vi "Serialize Properties.vi"(8 "error in (no error)":errorcluster, 10 "Properties":refnum<class "Property.lvclass">[](array[class]), 11 "Node in":refnum<k20>) -> (0 "error out":errorcluster, 3 "Node out":refnum<k20>)   [LabVIEW 2013, in "JUnit XML.lvlib" / "Test Suite.lvclass"]
uses:
  Test Suite.lvclass
  <vilib>/xml/NI_XML.lvlib
  JUnit XML.lvlib
  <vilib>/xml/Close Reference(Node).vi
  Property/Property.lvclass
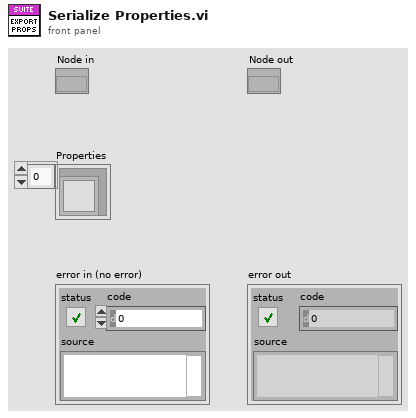
[diagram p1: front panel]
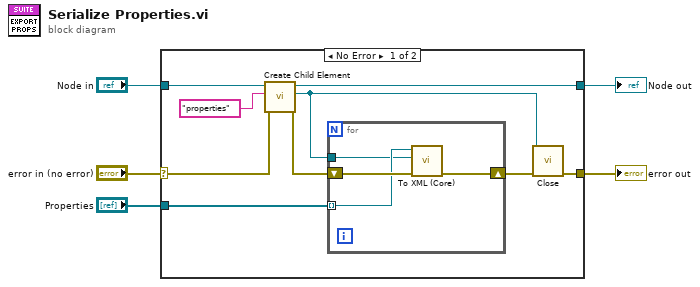
[diagram p0: block diagram]
diagram:
  n1 = case shown="No Error" "error in (no error)" {
    selector: "error in (no error)" -> [w7 w20]
    tunnel: "Node in" -> [w14 w19]
    tunnel: [w12 w20] -> w4
    tunnel: [w11 w19] -> w3
    tunnel: "Properties" -> [w9 _]
    frame No Error {
      n2 = call "Create Child Element.vi"("error in (no error)"=w7, "Name"="properties" ("Tag Name"), "Node in"=w14) -> ("error out"=w10:errorcluster, "Child Element"=w6:refnum<k20>, "Node out"=w11:refnum<k20>)  [unwired: 6 in]
      n3 = for {
        shift-right: [w18] -> w8
        shift-left: w10 -> [w17]
        tunnel: w9 -> [w16] mode=indexing
        tunnel: w6 -> [w15]
        n4 = call-dynamic "To XML (Core).vi"("error in (no error)"=w17, "Parent"=w15, "Property in"=w16) -> ("error out"=w18:errorcluster)  [unwired: 8 in]
      }
      n5 = call-poly <vilib>:"Close.vi"("error in (no error)"=w8, "node"=w6) -> ("error out"=w12:errorcluster)  [unwired: 7 in]
    }
    frame Error {
    }
  }
  "error out" <- w4
  "Node out" <- w3
